vi "RemoteVI Hide Remote Popups.vi"(0 "panel hWnd":u64, 1 "remote click?":bool, 5 "all popups":T1(array[cluster]), 7 "previous popup hWnds":u64[](array[numeric]), 9 "previously hidden":u64[](array[numeric])) -> (4 "popup hWnds":u64[](array[numeric]), 6 "hidden hWnds":u64[](array[numeric]))   [LabVIEW 2020, in "RemoteVI.lvlib"]
doc: "Hides the popups a REMOTE user opened (docs\\architecture.md, Popups): a popup in all popups that was not in previous popup hWnds is new; a new popup is hidden (RemoteVI Hide Window.vi, layered with alpha 0 - it stays open and clickable) when remote click? is TRUE (a client posted a button or key message within the last second), when a popup hidden before is still open (a submenu the remote hover opened with VK_RIGHT belongs to the remote user's menu, even long after the last click), and a new tip strip (class LVTipStrip) also when the host cursor is outside the panel window (RemoteVI Cursor Outside Window.vi) - it can only stem from the remote pointer. A popup in previously hidden is hidden again on every call while it is open, because a menu's fade-in animation sets its alpha back to 255 (measured). A popup opened at the host stays visible. Win32 only."
uses:
  RemoteVI.lvlib
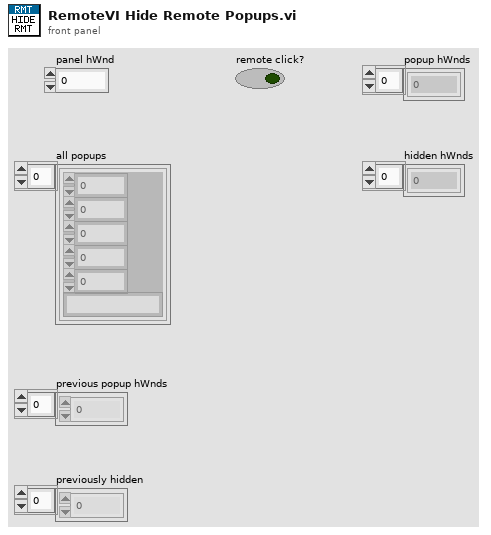
[diagram p1: front panel]
types:
  T1 = cluster{"hwnd":u64, "x":i32, "y":i32, "w":i32, "h":i32, "class":string}[]
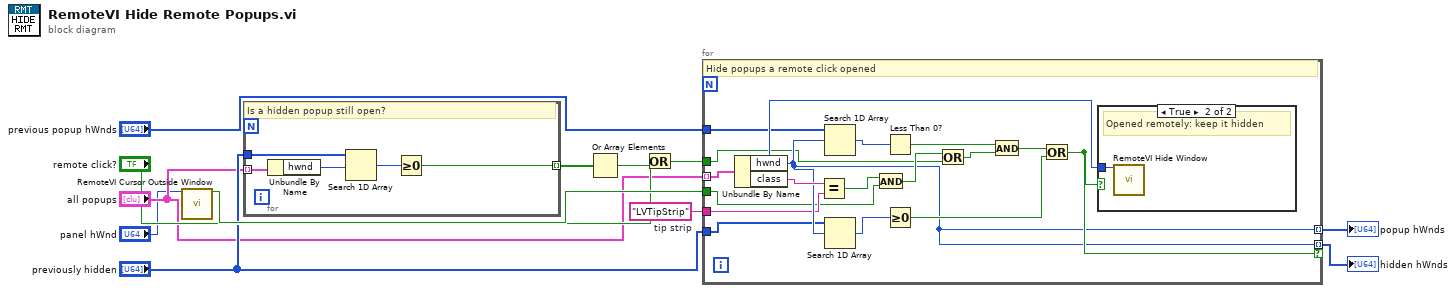
[diagram p0: block diagram]
diagram:
  w7 = "LVTipStrip"  # tip strip
  n1 = call "RemoteVI Cursor Outside Window.vi"("hWnd"="panel hWnd") -> ("outside?"=w6:bool)  [unwired: 14 in]
  n2 = for {
    tunnel: "all popups" -> [w13] mode=indexing
    tunnel: "previously hidden" -> [w14]
    tunnel: [w17] -> w8 mode=indexing
    # "Is a hidden popup still open?"
    n3 = Unbundle By Name(w13) -> ("hwnd"=w15:u64)
    n4 = Search 1D Array(1D array=w14, element=w15) -> (index of element=w16:i32)  [unwired: 1 in]
    n5 = Greater Or Equal To 0?(x=w16) -> (x >= 0?=w17:bool)
  }
  n6 = Or Array Elements(Boolean array=w8) -> (logical OR=w9:bool)
  n7 = Or(x="remote click?", y=w9) -> (x .or. y?=w10:bool)
  n8 = for {
    tunnel: "all popups" -> [w18] mode=indexing
    tunnel: "previous popup hWnds" -> [w19]
    tunnel: "previously hidden" -> [w21]
    tunnel: w7 -> [w23]
    tunnel: w6 -> [w22]
    tunnel: [w24] -> w11 mode=indexing
    tunnel: [w24] -> w12 mode=indexing if=w34
    tunnel: w10 -> [w20]
    # "Hide popups a remote click opened"
    n9 = Unbundle By Name(w18) -> ("hwnd"=w24:u64, "class"=w25:string)
    n10 = Equal?(x=w25, y=w23) -> (x = y?=w26:bool)
    n11 = Search 1D Array(1D array=w19, element=w24) -> (index of element=w29:i32)  [unwired: 1 in]
    n12 = Search 1D Array(1D array=w21, element=w24) -> (index of element=w32:i32)  [unwired: 1 in]
    n13 = And(x=w26, y=w22) -> (x .and. y?=w27:bool)
    n14 = Less Than 0?(x=w29) -> (x < 0?=w30:bool)
    n15 = Greater Or Equal To 0?(x=w32) -> (x >= 0?=w33:bool)
    n16 = Or(x=w27, y=w20) -> (x .or. y?=w28:bool)
    n17 = And(x=w30, y=w28) -> (x .and. y?=w31:bool)
    n18 = Or(x=w31, y=w33) -> (x .or. y?=w34:bool)
    n19 = case shown="True" w34 {
      tunnel: w24 -> [_ w35]
      frame False {
      }
      frame True {
        # "Opened remotely: keep it hidden"
        n20 = call "RemoteVI Hide Window.vi"("hwnd"=w35) -> ()  [unwired: 13 in, 2 out]
      }
    }
  }
  "popup hWnds" <- w11
  "hidden hWnds" <- w12
